vi "update Remote Display.vi"(8 "error in (no error)":errorcluster, 10 "Remote Display On?":bool, 11 "Keysight 9020A in":refnum<class "Keysight 9020A.lvclass">) -> (0 "error out":errorcluster, 3 "Keysight 9020A out":refnum<class "Keysight 9020A.lvclass">)   [LabVIEW 2023, in "Spectrum Analyzer.lvlib" / "Keysight 9020A.lvclass"]
uses:
  Keysight 9020A.lvclass
  Keysight 9020A.lvclass/Keysight 9020A.ctl
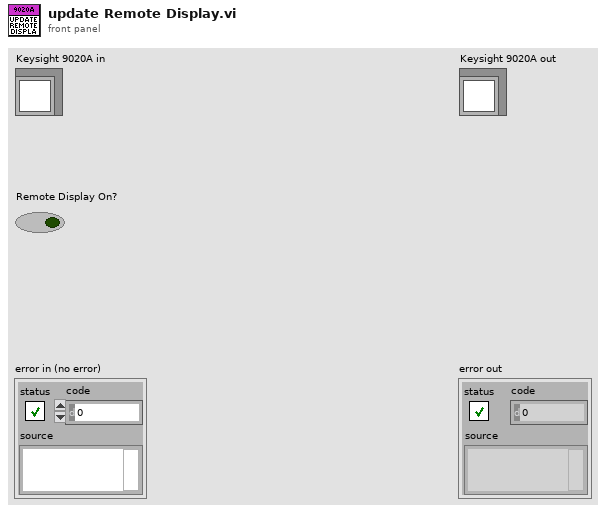
[diagram p1: front panel]
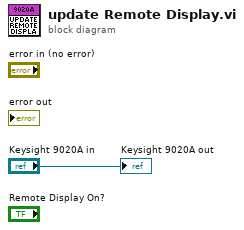
[diagram p0: block diagram]
diagram:
  "Keysight 9020A out" <- "Keysight 9020A in"
